vi "Handle MCP Request.vi"(4 "stream":string, 5 "Mcp-Name":string, 6 "Mcp-Method":string, 7 "parameters":string[][](array[string]), 8 "error in":errorcluster, 9 "protocol version":string, 10 "id in":i32, 11 "request":string) -> (0 "error out":errorcluster, 2 "status code":u16, 3 "response":string)   [LabVIEW 2020, in "MCP Server.lvlib"]
doc: "Handles the body of one HTTP POST in either MCP era and returns the HTTP status code and the response body. Replaces the direct call of Handle Server Request Batch.vi in Process HTTP Request.vi.\n\nERA, per request, without session state: a JSON object whose params._meta carries io.modelcontextprotocol/protocolVersion is MODERN (MCP 2026-07-28), unless its method is initialize. Everything else is LEGACY and is passed to Handle Server Request Batch.vi unchanged, so legacy answers stay exactly as they were.\n\nMODERN requests are checked first, in this order, and refused without being handled:\n- MCP-Protocol-Version header missing or different from the _meta protocolVersion: 400, -32020 (header mismatch).\n- protocolVersion not one of the modern versions of Supported Protocol Versions.vi: 400, -32022 with data.supported and data.requested.\n- Mcp-Method header missing or different from method: 400, -32020.\n- tools/call and prompts/get: Mcp-Name must equal params.name; resources/read: params.uri. A value =?base64?...?= is decoded first. Missing or different: 400, -32020.\n- io.modelcontextprotocol/clientCapabilities missing in params._meta: 400, -32602.\n- A method the modern era does not have (it has server/discover, tools/list, tools/call, prompts/list, prompts/get, resources/list, resources/read and resources/templates/list; no ping, logging/setLevel or notifications/initialized): 404, -32601. Notifications (no id) are answered with 202 as before.\nA JSON array (batch) that comes with modern headers (an Mcp-Method header, or a modern MCP-Protocol-Version) is refused with 400, -32600.\n\nMODERN results: server/discover is answered here (supportedVersions = all versions, capabilities and serverInfo as initialize reports them). Every other result is handled as before and then gets \"resultType\":\"complete\" and _meta io.modelcontextprotocol/serverInfo; the methods named in Cache Hints.vi also get ttlMs and cacheScope. resources/read errors -32002 (resource not found) become -32602.\n\nREQUEST CONTEXT: while a request is handled, its context ({\"era\",\"elicitation\",\"inputResponses\",\"id\",\"progressToken\",\"stream\"}) is the only element of the named queue \"MCP Request Context\" (size 1, which also serialises request handling), and questions that Ask User.vi registers are collected from the named queue \"MCP Input Requests\". When a modern tools/call registered questions, the result is {\"resultType\":\"input_required\",\"inputRequests\":{...}} instead of the tool result (no requestState: the retry carries the original params with inputResponses).\n\nserverInfo is taken from initialize.vi (called with a synthetic initialize request), so name and version always match what initialize reports.\n\nSTREAMING: stream is empty for a normal request. For a streamed tools/call Run Streamed Request.vi passes the stream object {\"events\":..,\"cancelled\":..} (the queues of the MCP SSE Response, as numbers); it goes into the request context, where Report Progress.vi and Cancel Requested.vi find it. id and progressToken in the context are the JSON text of the request id and of params._meta.progressToken."
uses:
  MCP Server.lvlib
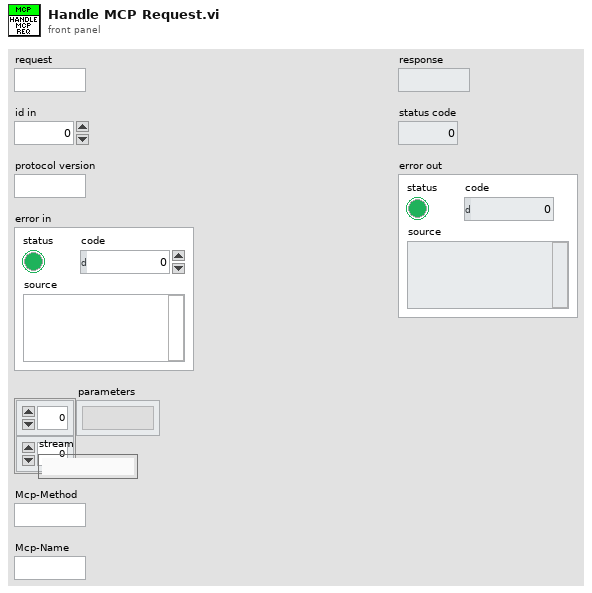
[diagram p1: front panel]
types:
  T1 = typedef "MCP Server.lvlib/MCP Request Metadata.ctl" = cluster{"method":string, "id":string, "has id":bool, "modern":bool, "discover":bool, "batch":bool, "protocol version":string, "client capabilities":bool, "name or uri":string, "elicitation":bool, "input responses":string}
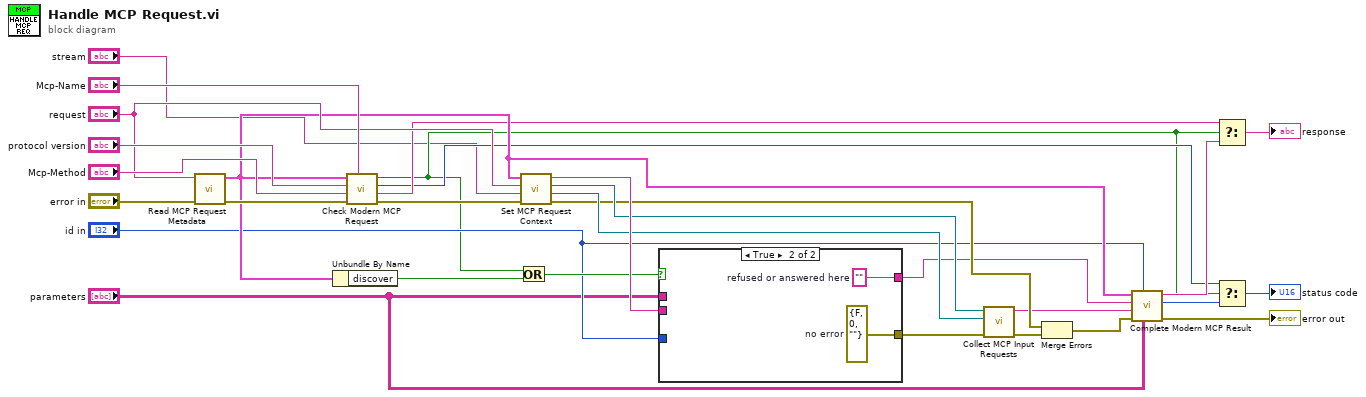
[diagram p0: block diagram]
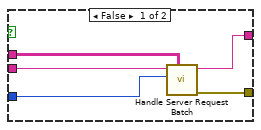
[diagram p2: hidden frame]
diagram:
  n1 = call "Read MCP Request Metadata.vi"("error in"="error in", "request"="request") -> ("error out"=w27:errorcluster, "MCP Request Metadata"=w15:T1)  [unwired: 8 in]
  n2 = Unbundle By Name(w15) -> ("discover"=w23:bool)
  n3 = call "Check Modern MCP Request.vi"("Mcp-Name"="Mcp-Name", "error in"=w27, "Mcp-Method"="Mcp-Method", "protocol version"="protocol version", "MCP Request Metadata"=w15) -> ("error out"=w24:errorcluster, "response"=w9:string, "status code"=w7:u16, "refused"=w6:bool)  [unwired: 3 in]
  n4 = Or(x=w6, y=w23) -> (x .or. y?=w21:bool)
  n5 = call "Set MCP Request Context.vi"("error in"=w24, "stream"="stream", "request"="request", "MCP Request Metadata"=w15) -> ("error out"=w17:errorcluster, "input requests queue"=w19:refnum<queue>, "context queue"=w20:refnum<queue>, "request out"=w22:string)  [unwired: 4 in]
  n6 = case shown="True" w21 {
    tunnel: w22 -> [w35 _]
    tunnel: "id in" -> [w34 _]
    tunnel: "parameters" -> [w33 _]
    tunnel: [w32 w37] -> w14
    tunnel: [w31 w36] -> w18
    frame False {
      n7 = call "Handle Server Request Batch.vi"("parameters"=w33, "id in"=w34, "request"=w35) -> ("error out"=w31:errorcluster, "response"=w32:string)  [unwired: 7 in]
    }
    frame True {
      w36 = errorcluster {"status"=FALSE, "code"=0, "source"=""}  # no error
      w37 = ""  # refused or answered here
    }
  }
  n8 = call "Collect MCP Input Requests.vi"("error in"=w18, "input requests queue"=w19, "context queue"=w20) -> ("error out"=w16:errorcluster, "input requests"=w13:string)  [unwired: 7 in]
  n9 = Merge Errors(w17, w16) -> (w12:errorcluster)
  n10 = call "Complete Modern MCP Result.vi"("parameters"="parameters", "id in"="id in", "error in"=w12, "input requests"=w13, "handler response"=w14, "MCP Request Metadata"=w15) -> ("error out"=→"error out":errorcluster, "status code"=w5:u16, "response"=w8:string)  [unwired: 3 in]
  n11 = Select(t=w9, s=w6, f=w8) -> (s? t:f=→"response":string)
  n12 = Select(t=w7, s=w6, f=w5) -> (s? t:f=→"status code":u16)
